vi "Determine Tx Msg.vi"(1 "Tx Msg Type":dbl format="%#_13g") -> (0 "Tx String":string)   [LabVIEW 2017]
uses:
  Tx Message Type.ctl
  Two Way Event Recorder Custom Device.lvlib
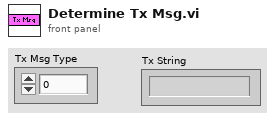
[diagram p1: front panel]
types:
  T1 = typedef "Two Way Event Recorder Custom Device.lvlib/Tx Message Type.ctl" = enum16{"Normal Time Stamp", "Time Stamp +30s", "Time Stamp -30s", "Malformed Data - Extra Character", "Malformed Data - Reduced Character", "Malformed Data - Invalid Characters"}
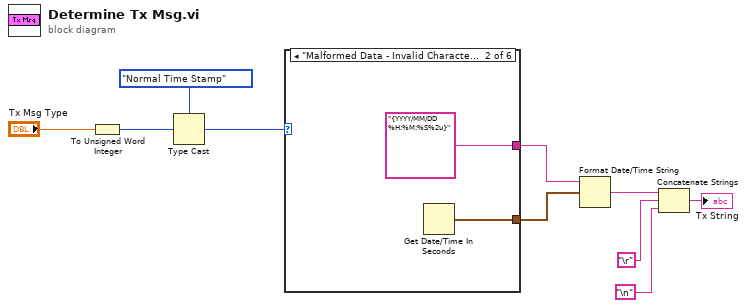
[diagram p0: block diagram]
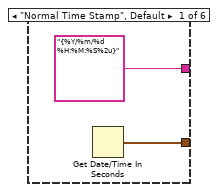
[diagram p2: hidden frame]
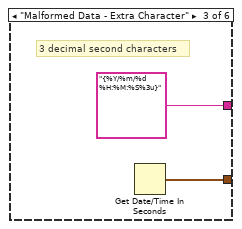
[diagram p3: hidden frame]
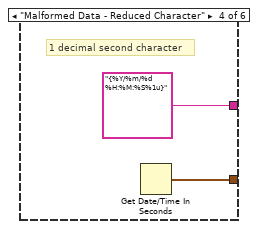
[diagram p4: hidden frame]
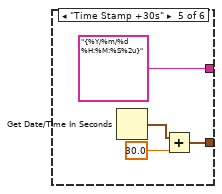
[diagram p5: hidden frame]
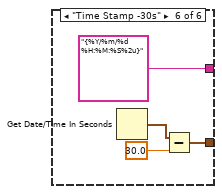
[diagram p6: hidden frame]
diagram:
  n1 = To Unsigned Word Integer(number="Tx Msg Type") -> (unsigned 16bit integer=w5:u16)
  n2 = Type Cast(type=Tx_Message_Type."Normal Time Stamp" ("Tx Message Type"), x=w5) -> (*(type *) &x=w7:T1)
  n3 = case shown="\"Malformed Data - Invalid Characters\"" w7 {
    tunnel: ["{%Y/%m/%d %H:%M:%S%2u}" ("time format string (%c)") "{YYYY/MM/DD %H:%M:%S%2u}" ("time format string (%c)") "{%Y/%m/%d %H:%M:%S%3u}" ("time format string (%c)") "{%Y/%m/%d %H:%M:%S%1u}" ("time format string (%c)") "{%Y/%m/%d %H:%M:%S%2u}" ("time format string (%c)") "{%Y/%m/%d %H:%M:%S%2u}" ("time format string (%c)")] -> w10
    tunnel: [w11 w13 w15 w17 w19 w23] -> w9
    frame "Normal Time Stamp", Default {
      n4 = Get Date/Time In Seconds() -> (seconds since 1Jan1904=w11:timestamp)
    }
    frame "Malformed Data - Invalid Characters" {
      n5 = Get Date/Time In Seconds() -> (seconds since 1Jan1904=w13:timestamp)
    }
    frame "Malformed Data - Extra Character" {
      # "3 decimal second characters"
      n6 = Get Date/Time In Seconds() -> (seconds since 1Jan1904=w15:timestamp)
    }
    frame "Malformed Data - Reduced Character" {
      # "1 decimal second character"
      n7 = Get Date/Time In Seconds() -> (seconds since 1Jan1904=w17:timestamp)
    }
    frame "Time Stamp +30s" {
      n8 = Get Date/Time In Seconds() -> (seconds since 1Jan1904=w20:timestamp)
      n9 = Add(x=w20, y=30.0) -> (x+y=w19:timestamp)
    }
    frame "Time Stamp -30s" {
      n10 = Get Date/Time In Seconds() -> (seconds since 1Jan1904=w24:timestamp)
      n11 = Subtract(x=w24, y=30.0) -> (x-y=w23:timestamp)
    }
  }
  n12 = Format Date/Time String(time format string (%c)=w10, seconds (now)=w9) -> (date/time string=w4:string)  [unwired: 1 in]
  n13 = Concatenate Strings(w4, "\r", "\n") -> (→"Tx String":string)
